vi "set UL_DL Center Channel Number.vi"(8 "error in (no error)":errorcluster, 9 "Direction":T1, 10 "Center Channel Argements":T2, 11 "NR in":refnum<class "NR.lvclass">) -> (0 "error out":errorcluster, 3 "NR out":refnum<class "NR.lvclass">)   [LabVIEW 2023, in "ANRITSU Call Box.lvlib" / "NR.lvclass"]
uses:
  NR.lvclass
  NR.lvclass/NR.ctl
  Type Definition/Uplink Downlink Enum.ctl
  ANRITSU Call Box.lvlib
  Type Definition/NR Center Channel Arguments.ctl
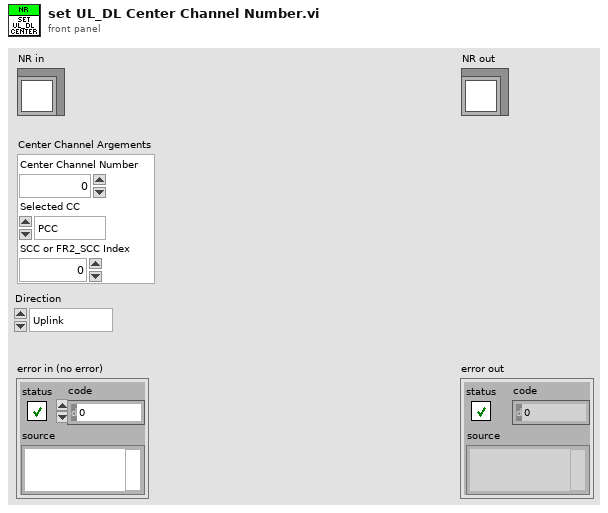
[diagram p1: front panel]
types:
  T1 = typedef "ANRITSU Call Box.lvlib/Uplink Downlink Enum.ctl" = enum16{"Uplink", "Downlink"}
  T2 = typedef "ANRITSU Call Box.lvlib/NR Center Channel Arguments.ctl" = cluster{"Center Channel Number":u32, "Selected CC":enum16{"PCC", "SCC", "FR2_PCC", "FR2_SCC"}, "SCC or FR2_SCC Index":u32}
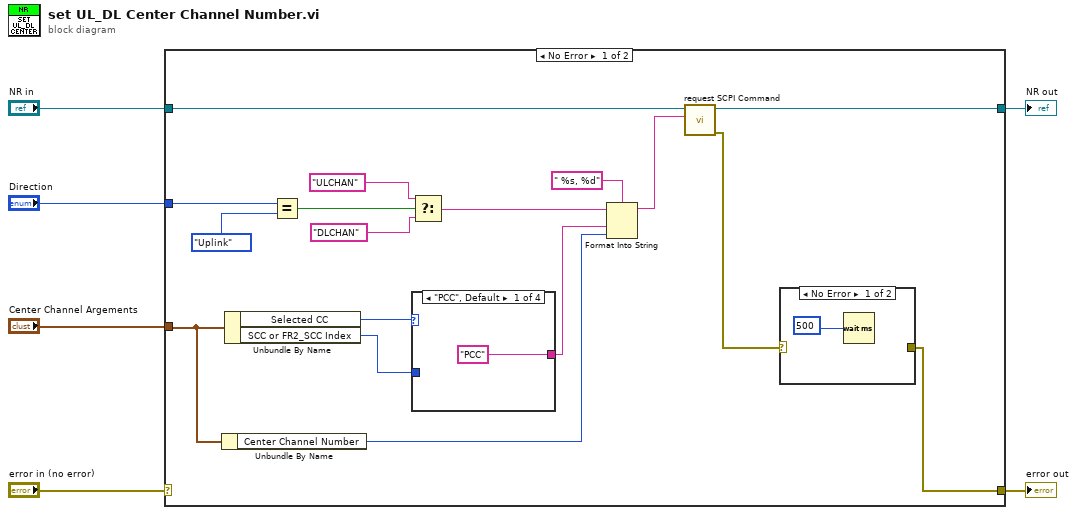
[diagram p0: block diagram]
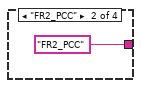
[diagram p3: hidden frame]
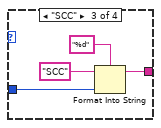
[diagram p4: hidden frame]
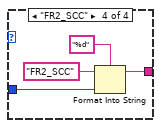
[diagram p5: hidden frame]
diagram:
  n1 = case shown="No Error" "error in (no error)" {
    selector: "error in (no error)" -> [_ w37]
    tunnel: [w7 w37] -> w5
    tunnel: [w10 w36] -> w3
    tunnel: "NR in" -> [w11 w36]
    tunnel: "Direction" -> [w23 _]
    tunnel: "Center Channel Argements" -> [w13 _]
    frame No Error {
      n2 = Unbundle By Name(w13) -> ("Center Channel Number"=w12:u32)
      n3 = Unbundle By Name(w13) -> ("Selected CC"=w18:enum16{"PCC", "SCC", "FR2_PCC", "FR2_SCC"}, "SCC or FR2_SCC Index"=w17:u32)
      n4 = Equal?(x=w23, y=Uplink_Downlink_Enum."Uplink") -> (x = y?=w19:bool)
      n5 = case shown="\"PCC\", Default" w18 {
        tunnel: ["PCC" "FR2_PCC" w28 w32] -> w14
        tunnel: w17 -> [_ _ w29 w33]
        frame "PCC", Default {
        }
        frame "FR2_PCC" {
        }
        frame "SCC" {
          n6 = Format Into String(format string="%d", initial string="SCC", w29) -> (resulting string=w28:string)  [unwired: 1 in, 1 out]
        }
        frame "FR2_SCC" {
          n7 = Format Into String(format string="%d", initial string="FR2_SCC", w33) -> (resulting string=w32:string)  [unwired: 1 in, 1 out]
        }
      }
      n8 = Select(t="ULCHAN", s=w19, f="DLCHAN") -> (s? t:f=w15:string)
      n9 = Format Into String(format string=" %s, %d", initial string=w15, w14, w12) -> (resulting string=w9:string)  [unwired: 1 in, 1 out]
      n10 = call "request SCPI Command.vi"("SCPI Command"=w9, "NR in"=w11) -> ("error out"=w8:errorcluster, "NR out"=w10:refnum<class "NR.lvclass">)  [unwired: 8 in]
      n11 = case shown="No Error" w8 {
        selector: w8 -> [_ w25]
        tunnel: [_ w25] -> w7
        frame No Error {
          n12 = Wait (ms)(milliseconds to wait=u32 500) -> ()  [unwired: 1 out]
        }
        frame Error {
        }
      }
    }
    frame Error {
    }
  }
  "error out" <- w5
  "NR out" <- w3
